vi "NextQ0FileData.vi"(8 "error in (no error)":errorcluster, 10 "Vfi":dbl[](array[numeric]), 11 "Scope5761 in":refnum<class "Scope5782_six_channel.lvclass">) -> (0 "error out":errorcluster, 2 "file data":dbl[][](array[numeric]), 3 "Scope5761 out":refnum<class "Scope5782_six_channel.lvclass">)   [LabVIEW 2025, in "Scope5782_six_channel.lvclass"]
uses:
  Scope5782_six_channel.lvclass
  Scope5782_six_channel.lvclass/Scope5782_six_channel.ctl
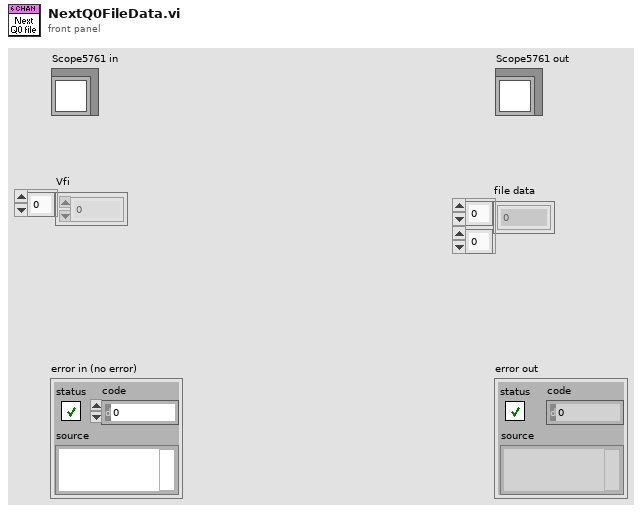
[diagram p1: front panel]
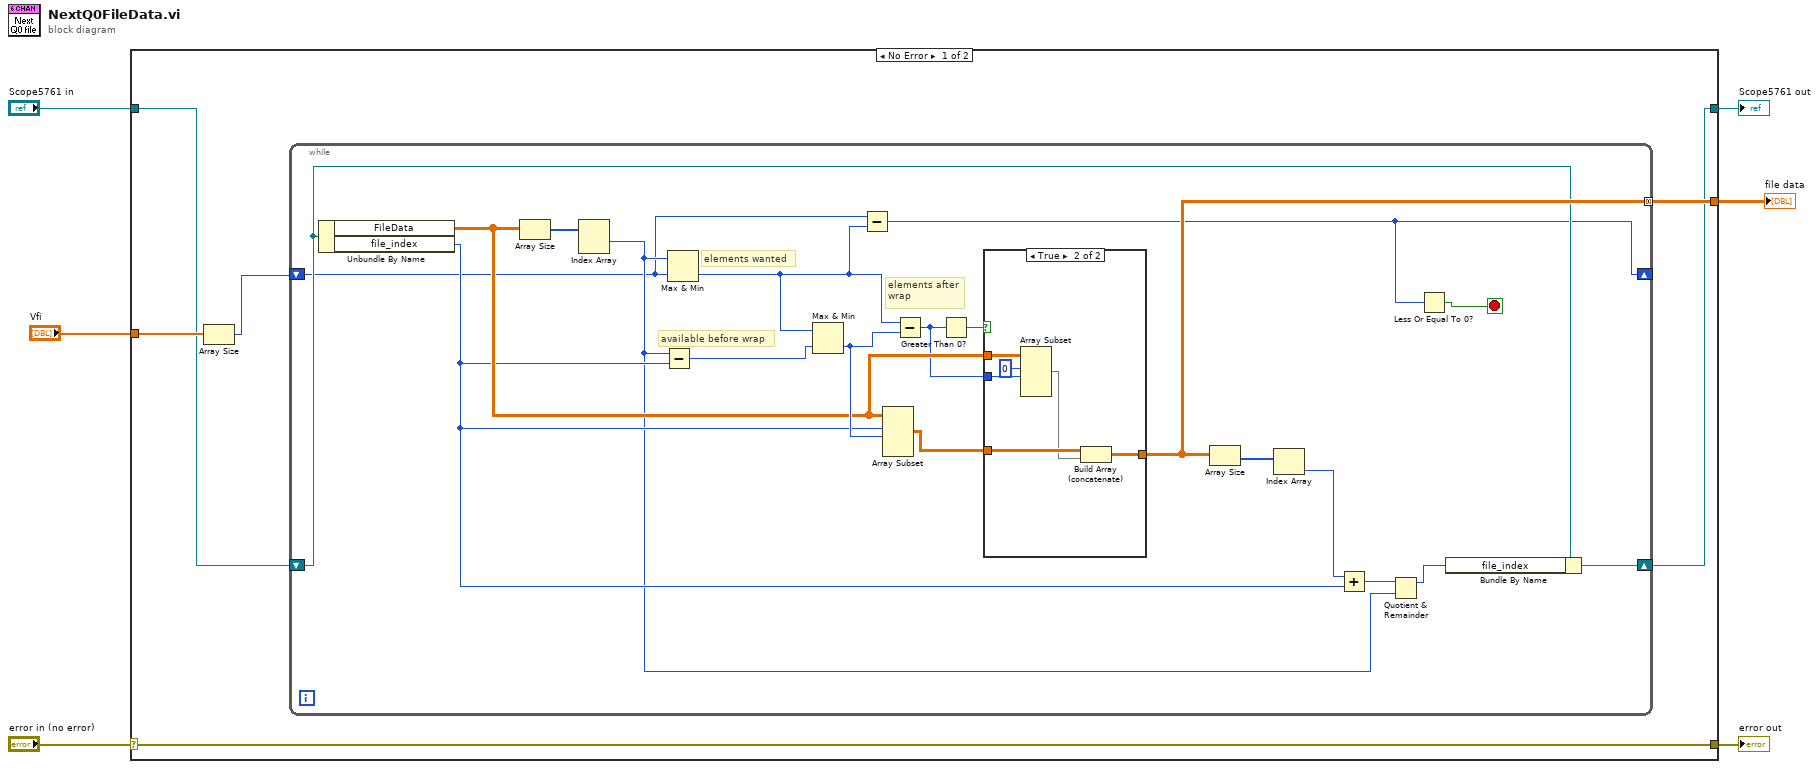
[diagram p0: block diagram]
diagram:
  n1 = case shown="No Error" "error in (no error)" {
    selector: "error in (no error)" -> [w12 w41]
    tunnel: [w12 w41] -> w5
    tunnel: [w7 w40] -> w3
    tunnel: "Scope5761 in" -> [w8 w40]
    tunnel: "Vfi" -> [w11 _]
    tunnel: [w9 _] -> w1
    frame No Error {
      n2 = Array Size(array=w11) -> (size(s)=w10:i32)
      n3 = while {
        tunnel: [w25] -> w9 mode=concatenating
        shift-right: [w18] -> w7
        shift-left: w8 -> [w17]
        shift-right: [w14] -> _
        shift-left: w10 -> [w16]
        stop <- w13 stop-if-true
        # "elements after\nwrap"
        # "elements wanted"
        # "available before wrap"
        n4 = Unbundle By Name(w17) -> ("FileData"=w29:dbl[][], "file_index"=w24:i32)
        n5 = Array Size(array=w29) -> (size(s)=w32:i32[])
        n6 = Index Array(array=w32) -> (element #1=w20:i32)  [unwired: 2 in, 1 out]
        n7 = Subtract(x=w20, y=w24) -> (x-y=w31:i32)
        n8 = Max & Min(x=w20, y=w16) -> (min(x,y)=w15:i32)  [unwired: 1 out]
        n9 = Max & Min(x=w15, y=w31) -> (min(x,y)=w30:i32)  [unwired: 1 out]
        n10 = Subtract(x=w16, y=w15) -> (x-y=w14:i32)
        n11 = Array Subset(array=w29, index (row)=w24, length (row)=w30) -> (w28:dbl[][])  [unwired: 2 in]
        n12 = Subtract(x=w15, y=w30) -> (x-y=w26:i32)
        n13 = Greater Than 0?(x=w26) -> (x > 0?=w27:bool)
        n14 = case shown="True" w27 {
          tunnel: w29 -> [_ w39]
          tunnel: w26 -> [_ w38]
          tunnel: w28 -> [w33 w36]
          tunnel: [w33 w34] -> w25
          frame False {
          }
          frame True {
            n15 = Array Subset(array=w39, index (row)=0 ("index"), length (row)=w38) -> (w35:dbl[][])  [unwired: 2 in]
            n16 = Build Array (concatenate)(w36, w35) -> (w34:dbl[][])
          }
        }
        n17 = Array Size(array=w25) -> (size(s)=w23:i32[])
        n18 = Index Array(array=w23) -> (element=w22:i32)  [unwired: 1 in]
        n19 = Add(x=w22, y=w24) -> (x+y=w21:i32)
        n20 = Quotient & Remainder(x=w21, y=w20) -> (x-y*floor(x/y)=w19:i32)  [unwired: 1 out]
        n21 = Less Or Equal To 0?(x=w14) -> (x <= 0?=w13:bool)
        n22 = Bundle By Name(cluster=w17, "file_index"=w19) -> (w18:refnum<class "Scope5782_six_channel.lvclass">)
      }
    }
    frame Error {
    }
  }
  "error out" <- w5
  "Scope5761 out" <- w3
  "file data" <- w1
